vi "Insert Entry.vi"(6 "Now":timestamp, 7 "Project Store in":refnum<class "Project Store.lvclass">, 8 "error in":errorcluster, 9 "Inserted Entry":T1, 10 "Original Entry":T1, 11 "Time Entry Store in":refnum<class "Time Entry Store.lvclass">) -> (0 "error out":errorcluster, 1 "Running Entry":T1, 2 "Pieces":T2, 3 "Time Entry Store out":refnum<class "Time Entry Store.lvclass">, 5 "Project Store out":refnum<class "Project Store.lvclass">)   [LabVIEW 2026]
doc: "Inserts a new time entry inside an existing one and saves the result. The original entry is split into up to three pieces, in time order: piece 1 is the original (same ID, same description) ending at the inserted Start Time; then the inserted entry with a new ID and its own project, task, times and description; then piece 3, a new ID with the original project and task, starting at the inserted End Time and ending at the original End Time, with an empty description. A piece of zero length is dropped, except that piece 3 of a RUNNING original (End Time 0) is always kept and stays running. When piece 1 is dropped the original is deleted (Delete Entry) before the other pieces are saved. Each piece is saved with Save Entry, so it is filed into the month file of its own Start Time.\n\nThe inserted time must lie inside the original: inserted Start Time at or after the original Start Time, inserted End Time at or before the original End Time (at or before Now for a running original), and inserted End Time after inserted Start Time. Otherwise error 5104 (Insert Entry: the inserted time must lie inside the original entry.) is returned and nothing is written. Nothing is written either when error in carries an error.\n\nInputs: Time Entry Store in; Project Store in (supplies the name labels written to the file); Original Entry; Inserted Entry (its ID is ignored); Now (used only for a running original); error in.\nOutputs: Time Entry Store out; Project Store out; Pieces (the saved entries in time order); Running Entry (piece 3 when the original was running, otherwise an empty entry); error out.\n\nGenerated by: Claude"
uses:
  Storage/Time Entry Store/Time Entry Store.lvclass
  Storage/Rows/Time Entry.ctl
  Storage/Project Store/Project Store.lvclass
  Storage/Rows/Time Entry List.ctl
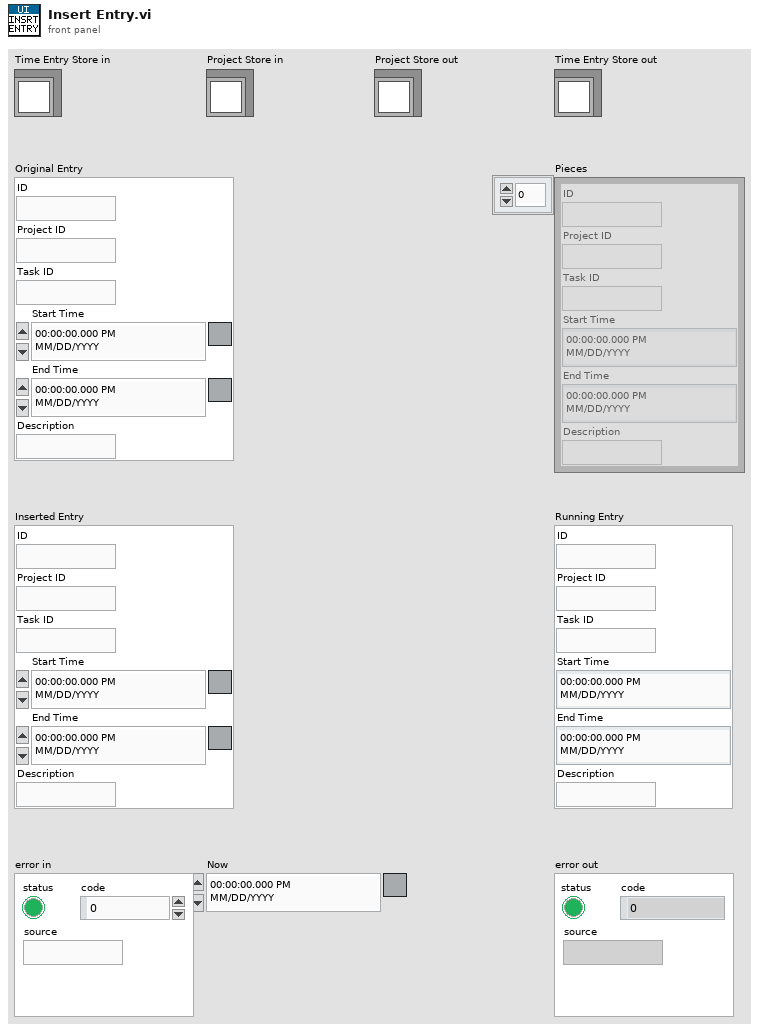
[diagram p1: front panel]
types:
  T1 = typedef "Time Entry.ctl" = cluster{"ID":string, "Project ID":string, "Task ID":string, "Start Time":timestamp, "End Time":timestamp, "Description":string}
  T2 = typedef "Time Entry List.ctl" = T1[]
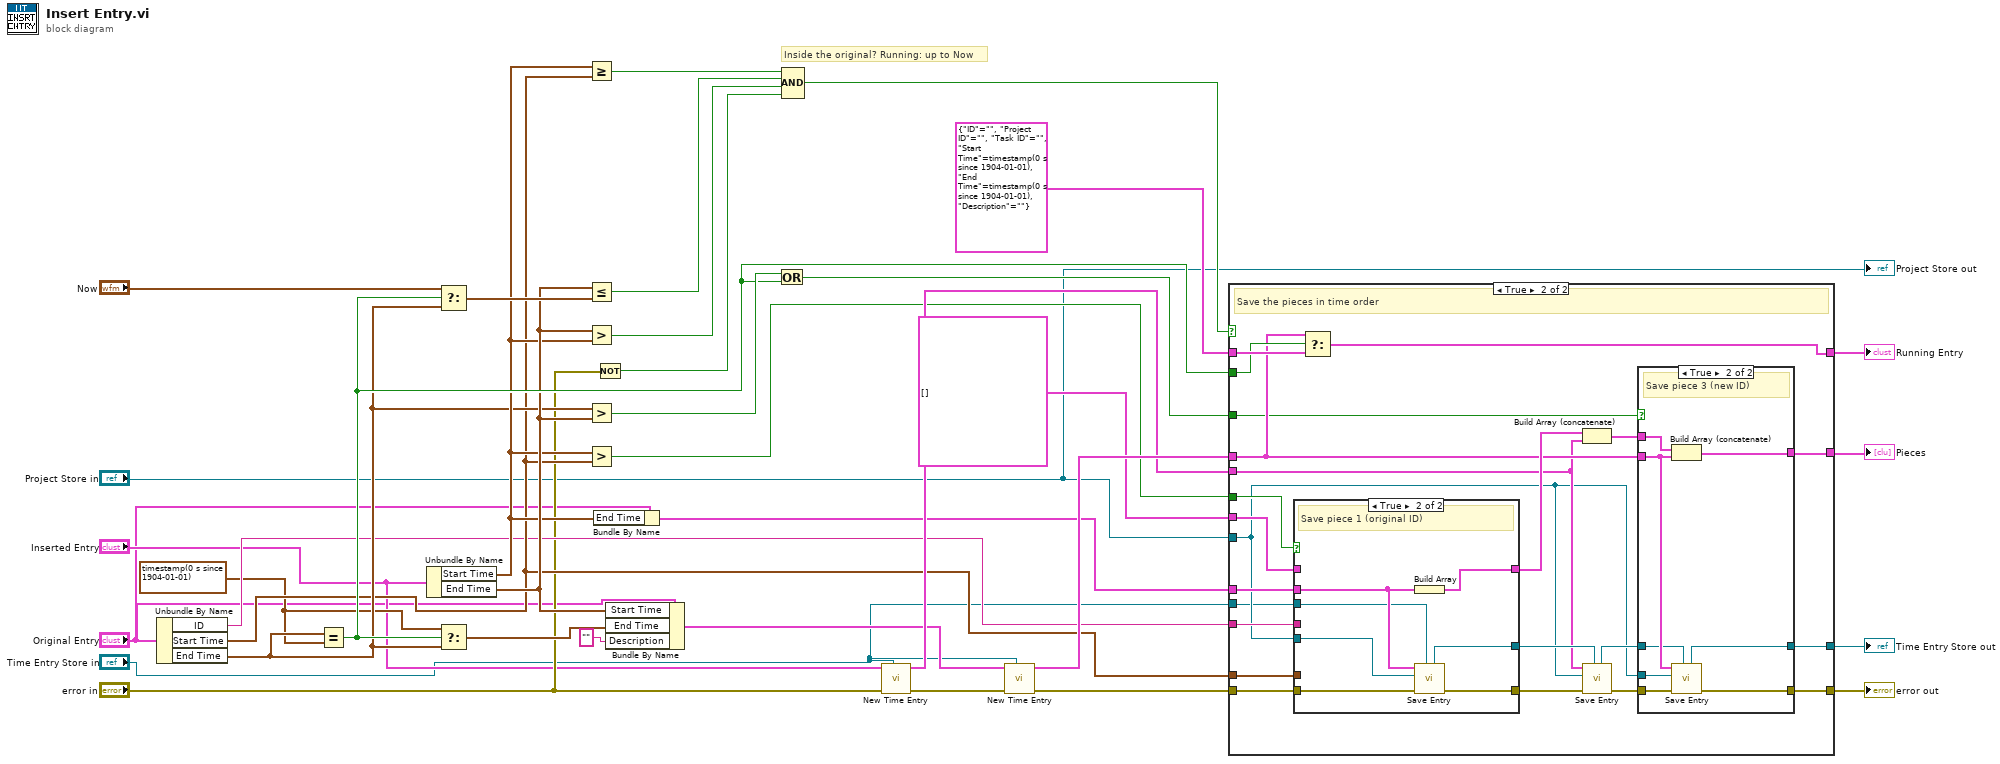
[diagram p0: block diagram]
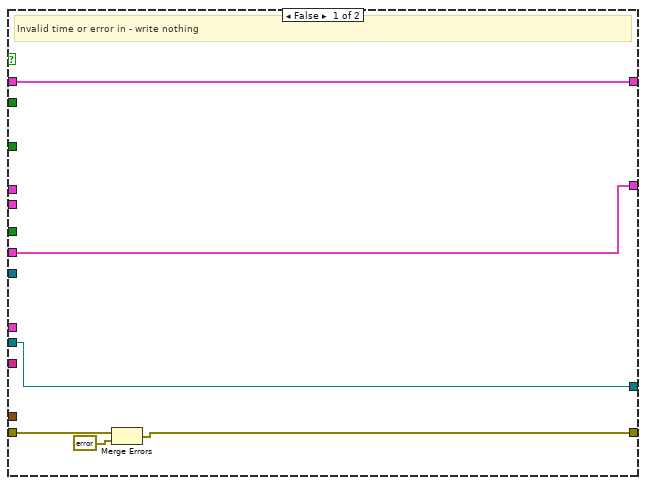
[diagram p2: hidden frame]
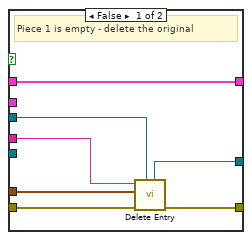
[diagram p4: hidden frame]
diagram:
  w11 = timestamp(0 s since 1904-01-01) ("still running")
  # "Inside the original? Running: up to Now"
  n1 = Unbundle By Name("Original Entry") -> ("ID"=w14:string, "Start Time"=w15:timestamp, "End Time"=w16:timestamp)
  n2 = Equal?(x=w16, y=w11) -> (x = y?=w19:bool)
  n3 = Unbundle By Name("Inserted Entry") -> ("Start Time"=w17:timestamp, "End Time"=w18:timestamp)
  n4 = Select(t="Now", s=w19, f=w16) -> (s? t:f=w20:timestamp)
  n5 = Select(t=w11, s=w19, f=w16) -> (s? t:f=w31:timestamp)
  n6 = Greater Or Equal?(x=w17, y=w15) -> (x >= y?=w21:bool)
  n7 = Less Or Equal?(x=w18, y=w20) -> (x <= y?=w22:bool)
  n8 = Greater?(x=w18, y=w17) -> (0:w23:bool)
  n9 = Greater?(x=w16, y=w18) -> (0:w27:bool)
  n10 = Greater?(x=w17, y=w15) -> (0:w26:bool)
  n11 = Bundle By Name(cluster="Original Entry", "End Time"=w17) -> (w30:T1)
  n12 = Not(x="error in") -> (.not. x?=w24:bool)
  n13 = Bundle By Name(cluster="Original Entry", "Start Time"=w18, "End Time"=w31, "Description"="" ("empty description")) -> (w32:T1)
  n14 = Or(x=w27, y=w19) -> (x .or. y?=w28:bool)
  n15 = Compound Arithmetic op=AND(w21, w22, w23, w24) -> (w25:bool)
  n16 = call "New Time Entry.vi"("Time Entry Store in"="Time Entry Store in", "error in (no error)"="error in", "Time Entry"="Inserted Entry") -> ("error out"=w34:errorcluster, "New Time Entry"=w33:T1)  [unwired: 6 in, 1 out]
  n17 = call "New Time Entry.vi"("Time Entry Store in"="Time Entry Store in", "error in (no error)"=w34, "Time Entry"=w32) -> ("error out"=w36:errorcluster, "New Time Entry"=w35:T1)  [unwired: 6 in, 1 out]
  n18 = case shown="True" w25 {
    tunnel: "Time Entry Store in" -> [w37 w43]
    tunnel: "Project Store in" -> [_ w44]
    tunnel: T2 [] ("no pieces") -> [w39 w54]
    tunnel: T1 {"ID"="", "Project ID"="", "Task ID"="", "Start Time"=timestamp(0 s since 1904-01-01), "End Time"=timestamp(0 s since 1904-01-01), "Description"=""} ("empty entry") -> [w40 w55]
    tunnel: w33 -> [_ w49]
    tunnel: w14 -> [_ w51]
    tunnel: w15 -> [_ w52]
    tunnel: [w37 w62] -> w7
    tunnel: [w39 w64] -> w8
    tunnel: [w40 w65] -> w9
    tunnel: w26 -> [_ w46]
    tunnel: w30 -> [_ w48]
    tunnel: w19 -> [_ w53]
    tunnel: w28 -> [_ w47]
    tunnel: w36 -> [w38 w45]
    tunnel: w35 -> [_ w50]
    tunnel: [w42 w63] -> w10
    frame False {
      # "Invalid time or error in - write nothing"
      n19 = Merge Errors(w38, errorcluster {"status"=TRUE, "code"=5104, "source"="Insert Entry: the inserted time must lie inside the original entry."} ("error 5104")) -> (w42:errorcluster)
    }
    frame True {
      # "Save the pieces in time order"
      n20 = case shown="True" w46 {
        tunnel: w43 -> [w77 w84]
        tunnel: w44 -> [_ w87]
        tunnel: w54 -> [w81 _]
        tunnel: w51 -> [w79 _]
        tunnel: w52 -> [w80 _]
        tunnel: [w81 w90] -> w58
        tunnel: w48 -> [_ w86]
        tunnel: w45 -> [w78 w85]
        tunnel: [w82 w88] -> w56
        tunnel: [w83 w89] -> w57
        frame False {
          # "Piece 1 is empty - delete the original"
          n21 = call-dynamic "Delete Entry.vi"("Time Entry Store in"=w77, "error in (no error)"=w78, "Start Time"=w80, "ID"=w79) -> ("error out"=w83:errorcluster, "Time Entry Store out"=w82:refnum<class "Time Entry Store.lvclass">)  [unwired: 5 in, 1 out]
        }
        frame True {
          # "Save piece 1 (original ID)"
          n22 = Build Array(w86) -> (w90:T1[])
          n23 = call-dynamic "Save Entry.vi"("Time Entry Store in"=w84, "error in (no error)"=w85, "Project Store"=w87, "Time Entry"=w86) -> ("error out"=w89:errorcluster, "Time Entry Store out"=w88:refnum<class "Time Entry Store.lvclass">)  [unwired: 6 in]
        }
      }
      n24 = Select(t=w50, s=w53, f=w55) -> (s? t:f=w65:T1)
      n25 = Build Array (concatenate)(w58, w49) -> (w61:T2)
      n26 = call-dynamic "Save Entry.vi"("Time Entry Store in"=w56, "error in (no error)"=w57, "Project Store"=w44, "Time Entry"=w49) -> ("error out"=w60:errorcluster, "Time Entry Store out"=w59:refnum<class "Time Entry Store.lvclass">)  [unwired: 6 in]
      n27 = case shown="True" w47 {
        tunnel: w44 -> [_ w72]
        tunnel: w61 -> [w68 w73]
        tunnel: [w68 w76] -> w64
        tunnel: w50 -> [_ w71]
        tunnel: w59 -> [w66 w69]
        tunnel: w60 -> [w67 w70]
        tunnel: [w66 w74] -> w62
        tunnel: [w67 w75] -> w63
        frame False {
          # "Piece 3 is empty - drop it"
        }
        frame True {
          # "Save piece 3 (new ID)"
          n28 = Build Array (concatenate)(w73, w71) -> (w76:T2)
          n29 = call-dynamic "Save Entry.vi"("Time Entry Store in"=w69, "error in (no error)"=w70, "Project Store"=w72, "Time Entry"=w71) -> ("error out"=w75:errorcluster, "Time Entry Store out"=w74:refnum<class "Time Entry Store.lvclass">)  [unwired: 6 in]
        }
      }
    }
  }
  "Time Entry Store out" <- w7
  "Pieces" <- w8
  "Running Entry" <- w9
  "error out" <- w10
  "Project Store out" <- "Project Store in"
